vi "PicoScope5000aGetValuesOverlapped.vi"(5 "Segment Range":T1 {"toSegmentIndex" format="%.4p"; "fromSegmentIndex" format="%.4p"}, 7 "Buffer and Transfer Settings":T2 {"Down-Sample Mode" items=["None", "Aggregate", "Decimate", "Average"]; "Down Sample Ratio" step=1; "Samples" format="%_6p"}, 8 "error in (no error)":errorcluster, 11 "handle in":i16) -> (0 "error out":errorcluster, 3 "handle out":i16, 4 "overflow":i16 format="%010b", 6 "noOfSamples":u64)   [LabVIEW 2009]
doc: "Calls ps5000aGetValuesOverlapped"
uses:
  ps5000a.dll
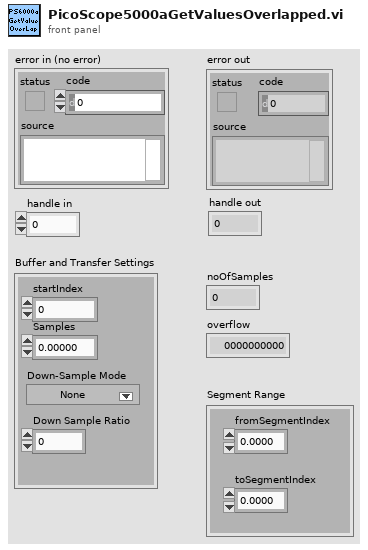
[diagram p1: front panel]
types:
  T1 = cluster{"fromSegmentIndex":u64, "toSegmentIndex":u64}
  T2 = cluster{"startIndex":u64, "Samples":u64, "Down Sample Ratio":u64, "Down-Sample Mode":u32}
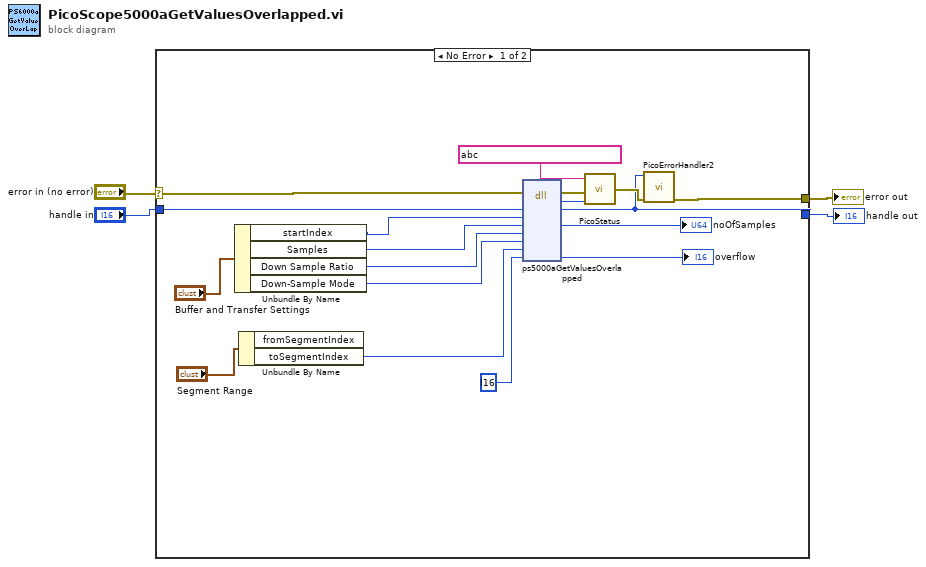
[diagram p0: block diagram]
diagram:
  n1 = case shown="No Error" "error in (no error)" {
    selector: "error in (no error)" -> [w12 w23]
    tunnel: "handle in" -> [w11 w24]
    tunnel: [w9 w24] -> w4
    tunnel: [w10 w23] -> w3
    frame #0 {
      n2 = Unbundle By Name("Buffer and Transfer Settings") -> ("startIndex"=w13:u64, "Samples"=w22:u64, "Down Sample Ratio"=w19:u64, "Down-Sample Mode"=w20:u32)
      n3 = Unbundle By Name("Segment Range") -> ("toSegmentIndex"=w6:u64)  [unwired: 1 out]
      n4 = dll-call lib="ps5000a.dll" fn="ps5000aGetValuesOverlapped" ("ps3000.dll:_ps3000_open_unit@0")(error in=w12, "handle"=w11, "startIndex"=w13, "noOfSamples"=w22, "downSampleRatio"=w19, "downSampleRatioMode"=w20, "segmentIndex"=w6, "overflow"=i16 ?) -> (error out=w18:errorcluster, "PICO_STATUS"=w17:u32, "handle"=w9:i16, "noOfSamples"=→"noOfSamples":u32, "overflow"=→"overflow":i16)  [unwired: 6 in, 1 out]
      n5 = call "PicoStatus.vi"("PICO STATUS"=w17, "error in"=w18, "source"=string ?) -> ("error out"=w21:errorcluster)
      n6 = call "PicoErrorHandler2.vi"("error in (no error)"=w21, "handle In"=w9) -> ("error out"=w10:errorcluster)  [unwired: 9 in]
    }
    frame #1 {
    }
  }
  "error out" <- w3
  "handle out" <- w4
